vi "Read Msg Input.vi"(11 "Stop Msg Input in":refnum<class "Stop Msg Input.lvclass">) -> (1 "Parent Stopped":bool, 2 "Safe Stop":bool=TRUE, 4 "Teller":refnum<class "Teller.lvclass">)   [LabVIEW 2020, in "jettl.lvlib" / "Stop jettl Msg.lvlib" / "Stop Msg Input.lvlib" / "Stop Msg Input.lvclass"]
uses:
  Stop Msg Input.lvclass
  Teller/Teller.lvclass
  Stop Msg Input.lvclass/Stop Msg Input.ctl
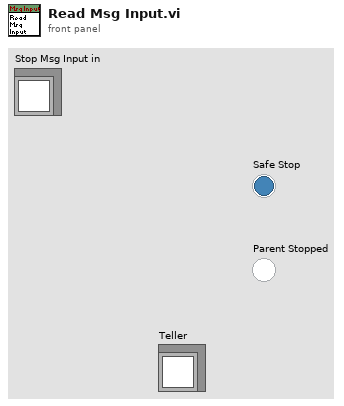
[diagram p1: front panel]
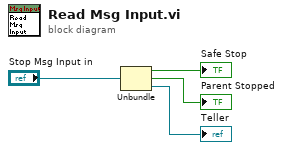
[diagram p0: block diagram]
diagram:
  n1 = Unbundle "Unbundle"("Stop Msg Input in") -> (→"Safe Stop":bool, →"Parent Stopped":bool, →"Teller":refnum<class "Teller.lvclass">)
